vi "Error Cluster From Error Code (Merecs).vi"(4 "is warning? (False)":bool, 5 "show call chain? (False)":bool, 6 "error in (no error)":errorcluster, 7 "error arguments (\"\")":string, 8 "error description (\"\")":string, 9 "error code (0)":i32) -> (0 "error out":errorcluster)   [LabVIEW 2019, in "Error Generation.lvlib"]
doc: "Converts an error or warning code to an error cluster. This VI is useful when you receive a return value from a shared library call or when you return user-defined error codes.\n\n<b>Original help for Error Cluster From Error Code.vi:</b>\n- - -\nCopyright (c) 2023, Merecs Engineering GmbH"
uses:
  Error Generation.lvlib
panel:
  in  "call chain header":string="<b>call chain</b>"
  # "\\n at the beginning removed"
  # "Connector Pane"
  # "Locals"
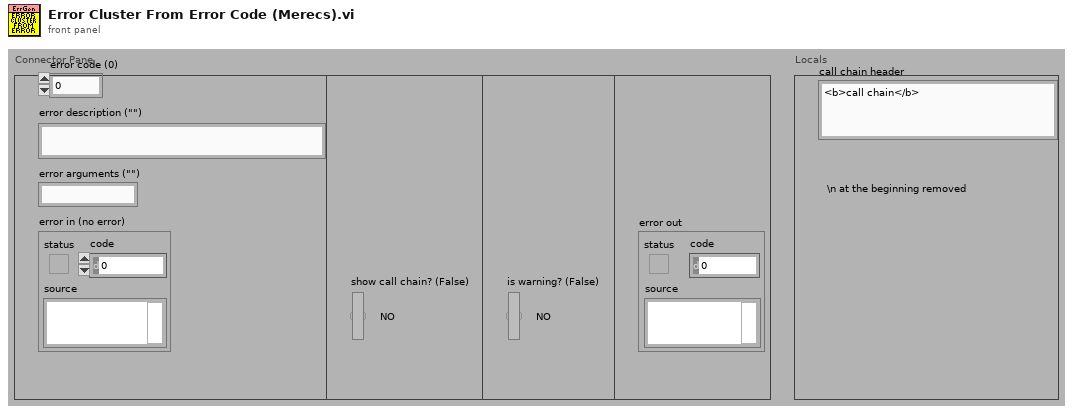
[diagram p1: front panel]
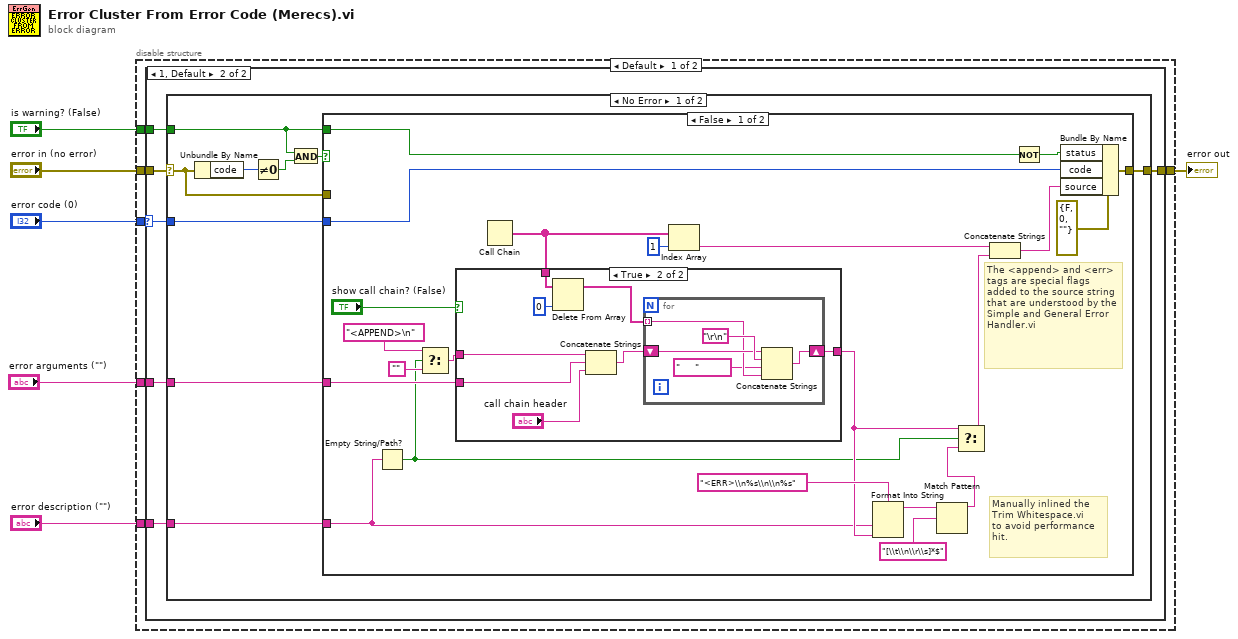
[diagram p0: block diagram]
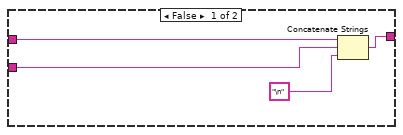
[diagram p3: hidden frame]
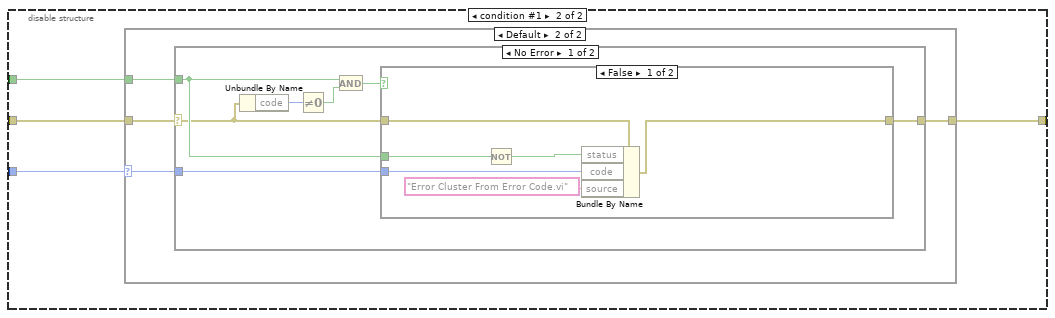
[diagram p6: hidden frame]
diagram:
  n1 = disable-structure shown="Default" {
    disable-tunnel: [w12 w72] -> w6
    disable-tunnel: "error in (no error)" -> [w11 w73]
    disable-tunnel: "error code (0)" -> [w10 w71]
    disable-tunnel: "error description (\"\")" -> [w9 _]
    disable-tunnel: "is warning? (False)" -> [w8 w70]
    disable-tunnel: "error arguments (\"\")" -> [w7 _]
    frame condition #0 (active) {
      n2 = case shown="1, Default" w10 {
        selector: w10 -> [_ w17]
        tunnel: [w13 w19] -> w12
        tunnel: w11 -> [w13 w18]
        tunnel: w9 -> [_ w16]
        tunnel: w8 -> [_ w15]
        tunnel: w7 -> [_ w14]
        frame 0 {
          # "If the error code in equals zero, then propagate the error in cluster regardless of its value."
        }
        frame 1, Default {
          n3 = case shown="No Error" w18 {
            selector: w18 -> [w23 w69]
            tunnel: [w28 w69] -> w19
            tunnel: w17 -> [w27 _]
            tunnel: w16 -> [w22 _]
            tunnel: w15 -> [w21 _]
            tunnel: w14 -> [w20 _]
            frame No Error {
              n4 = Unbundle By Name(w23) -> ("code"=w26:i32)
              n5 = Not Equal To 0?(x=w26) -> (x != 0?=w24:bool)
              n6 = And(x=w21, y=w24) -> (x .and. y?=w25:bool)
              n7 = case shown="False" w25 {
                tunnel: [w50 w68] -> w28
                tunnel: w27 -> [w46 _]
                tunnel: w23 -> [_ w68]
                tunnel: w21 -> [w43 _]
                tunnel: w22 -> [w38 _]
                tunnel: w20 -> [w33 _]
                frame False {
                  # "Manually inlined the\nTrim Whitespace.vi\nto avoid performance\nhit."
                  # "The <append> and <err> tags are special flags added to the source string that are understood by the Simple and General Error Handler.vi"
                  n8 = Empty String/Path?(string/path=w38) -> (empty?=w30:bool)
                  n9 = Select(t="<APPEND>\n", s=w30, f="") -> (s? t:f=w29:string)
                  n10 = Call Chain() -> (call chain=w44:string[])
                  n11 = case shown="True" "show call chain? (False)" {
                    tunnel: [w54 w62] -> w40
                    tunnel: w44 -> [_ w60]
                    tunnel: w29 -> [w51 w55]
                    tunnel: w33 -> [w53 w56]
                    frame False {
                      n12 = Concatenate Strings(w51, w53, "\n") -> (w54:string)
                    }
                    frame True {
                      n13 = Delete From Array(array=w60, index=0) -> (array with subset deleted=w59:string[])  [unwired: 1 in, 1 out]
                      n14 = Concatenate Strings(w55, w56, "call chain header") -> (w57:string)
                      n15 = for {
                        tunnel: w59 -> [w64] mode=indexing
                        shift-right: [w67] -> w62
                        shift-left: w57 -> [w65]
                        n16 = Concatenate Strings(w65, "\r\n", "     ", w64) -> (w67:string)
                      }
                    }
                  }
                  n17 = Index Array(array=w44, index=1) -> (element=w34:string)
                  n18 = Format Into String(format string="<ERR>\\n%s\\n\\n%s", w38, w40) -> (resulting string=w36:string)  [unwired: 2 in, 1 out]
                  n19 = Match Pattern(string=w36, regular expression="[\\t\\n\\r\\s]*$") -> (before substring=w35:string)  [unwired: 1 in, 3 out]
                  n20 = Select(t=w40, s=w30, f=w35) -> (s? t:f=w39:string)
                  n21 = Concatenate Strings(w34, w39) -> (w48:string)
                  n22 = Not(x=w43) -> (.not. x?=w47:bool)
                  n23 = Bundle By Name(cluster=errorcluster {"status"=FALSE, "code"=0, "source"=""} ("error out"), "status"=w47, "code"=w46, "source"=w48) -> (w50:errorcluster)
                }
                frame True {
                  # "If the error code input is setting a warning, and a warning is already set on the wire, then we\ngo with the one already on the wire."
                }
              }
            }
            frame Error {
              # "An error in trumps any error code input."
            }
          }
        }
      }
    }
    frame condition #1 {
      n24 = case shown="Default" w71 {
        selector: w71 -> [_ w76]
        tunnel: w73 -> [w74 w78]
        tunnel: [w74 w77] -> w72
        tunnel: w70 -> [_ w75]
        frame 0 {
          # "If the error code in equals zero, then propagate the error in cluster regardless of its value."
        }
        frame Default {
          n25 = case shown="No Error" w78 {
            selector: w78 -> [w80 w93]
            tunnel: [w84 w93] -> w77
            tunnel: w76 -> [w85 _]
            tunnel: w75 -> [w81 _]
            frame No Error {
              n26 = Unbundle By Name(w80) -> ("code"=w83:i32)
              n27 = Not Equal To 0?(x=w83) -> (x != 0?=w82:bool)
              n28 = And(x=w81, y=w82) -> (x .and. y?=w79:bool)
              n29 = case shown="False" w79 {
                tunnel: w85 -> [w91 _]
                tunnel: [w88 w92] -> w84
                tunnel: w81 -> [w87 _]
                tunnel: w80 -> [w86 w92]
                frame False {
                  n30 = Not(x=w87) -> (.not. x?=w90:bool)
                  n31 = Bundle By Name(cluster=w86, "status"=w90, "code"=w91, "source"="Error Cluster From Error Code.vi") -> (w88:errorcluster)
                }
                frame True {
                  # "If the error code input is setting a warning, and a warning is already set on the wire, then we\ngo with the one already on the wire."
                }
              }
            }
            frame Error {
              # "An error in trumps any error code input."
            }
          }
        }
      }
    }
  }
  "error out" <- w6
